vi "Consumer.vi"(8 "error in (no error)":errorcluster, 9 "Data":variant, 10 "Case ID":string, 11 "uService Template in":refnum<class "Common GUI v3.lvclass">) -> (0 "error out":errorcluster, 3 "uService Template out":refnum<class "Common GUI v3.lvclass">)   [LabVIEW 2020, in "TALOS.lvlib" / "Common GUI v3.lvlib" / "Common GUI v3.lvclass"]
uses:
  Common GUI v3.lvclass
  C:/LabVIEW Code/TALOS/talos/Ancestor/Ancestor/Ancestor.lvclass
  Common GUI v3 Consumer Case Selector.ctl
  Classes/Guardian List/Guardian List.lvclass
  Common GUI v3.lvclass/Common GUI v3.ctl
  Ancestor/Ancestor/Ancestor.lvclass/Ancestor.ctl
  Error Listbox Msg.ctl
  Error Listbox Msg Action.ctl
  Error Manager/Error Info.ctl
  Remote uService GUI.ctl
  Classes/uService List/uService List.lvclass/uService List.ctl
  Classes/uService List/Get Remote GUI.vi
  Classes/uService List/Get Remote Window VI Ref.vi
  Classes/uService List/Set Remote Window VI Ref.vi
  Classes/uService List/Get VI Ref.vi
  Support VIs/Generate Error.vi
  FGV/Error Memory/Get Error Description.vi
  Support VIs/Get PC name.vi
  Ancestor/Ancestor/Read ID.vi
  Support VIs/Get Class Name.vi
  <vilib>/Utility/error.llb/Clear Errors.vi
  FGV/Error Memory/Error Memory Core.vi
  <vilib>/AdvancedString/Delimited String to 1D String Array.vi
  Support VIs/Circus Root Path.vi
  FGV/Error Memory/Error Crt Lvl checker.vi
  FGV/Error Memory/Error Memory Core.vi/40c8088d-b597-4017-91af-faa98e00292e.vi
  FGV/Error Memory/Error Memory Core.vi/d4a3ab98-063c-4e44-b43d-fbdcfe6c2be2.vi
  Support VIs/Global Memory.vi
  <vilib>/Utility/LVClass/Get LV Class Name.vi
  Support VIs/Is in Packed Library.vi
  Support VIs/TALOS Root path.vi
  Support VIs/Read CSV worksheet.vi
  Support VIs/Global Constants.vi
  <vilib>/Utility/error.llb/General Error Handler.vi
  Support VIs/Error Log.vi
  Ancestor/Ancestor/Ancestor.lvclass
  <vilib>/Comparison/Equal/Equal Functor/Equal Functor.lvclass
  Classes/uService List/uService List.lvclass
  Father of all uServices/Father of all uServices/Father of all uServices.lvclass
  TALOS.lvlib
  Error Manager/Error Manager.lvclass
  Common GUI v3.lvlib
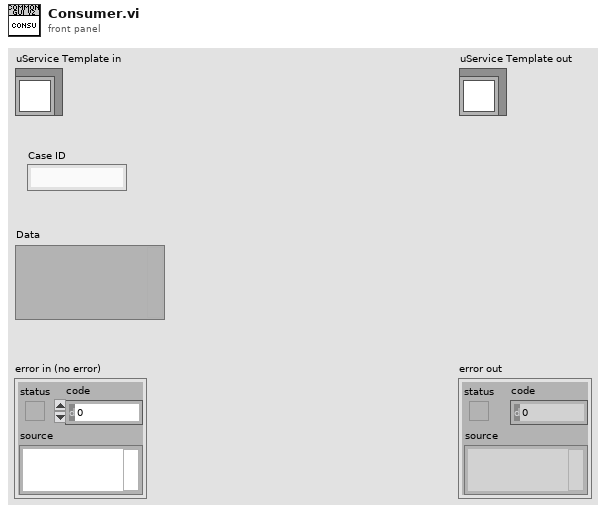
[diagram p1: front panel]
types:
  T1 = typedef "TALOS.lvlib/Common GUI v3.lvlib/Common GUI v3.lvclass/Common GUI v3 Consumer Case Selector.ctl" = enum16{"Update Guardians List", "Update ABORT LED", "Update Guardian ID", "Update Kasli Log", "Update Error Listbox", "Update Run Number", "Change Run LED color", "Update Run Status", "Run Stopped with Errors", "Reset Run LED", "Update Run Config", "Remote GUI"}
  T2 = typedef "TALOS.lvlib/Common GUI v3.lvlib/Common GUI v3.lvclass/Error Listbox Msg.ctl" = cluster{"Action":T3, "Error Info":T4}
  T3 = typedef "TALOS.lvlib/Common GUI v3.lvlib/Common GUI v3.lvclass/Error Listbox Msg Action.ctl" = enum16{"Add", "Remove", "Clear"}
  T4 = typedef "TALOS.lvlib/Error Manager.lvlib/Error Manager.lvclass/Error Info.ctl" = cluster{"error out":errorcluster, "Time Stamp":timestamp, "Machine Name":string, "GUID":string}
  T5 = typedef "TALOS.lvlib/Common GUI v3.lvlib/Remote uService GUI.ctl" = cluster{"Open/Close":bool, "uService ID":string}
  T6 = map{string, cluster{"Online":bool, "Last Poke":timestamp}}
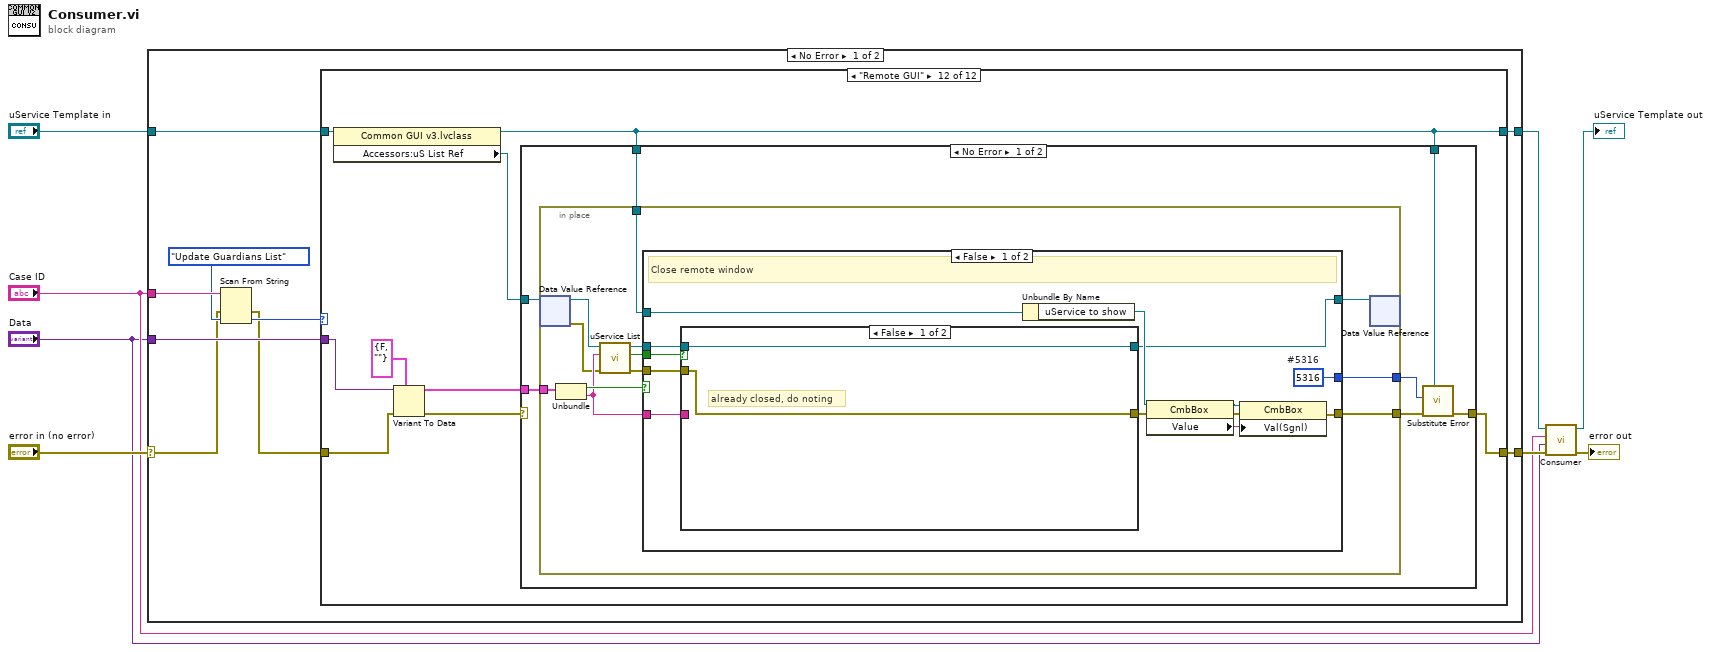
[diagram p0: block diagram]
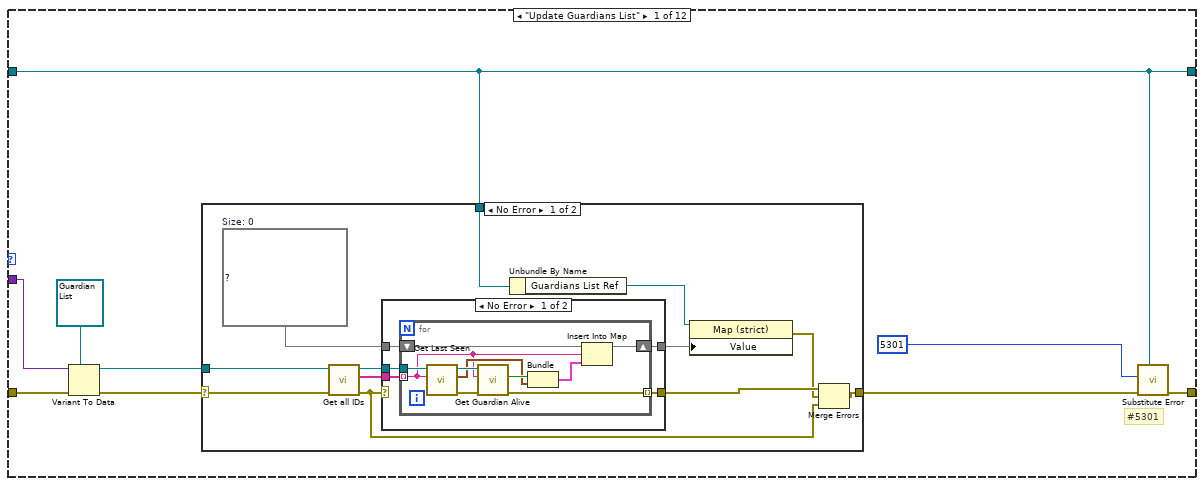
[diagram p2: hidden frame]
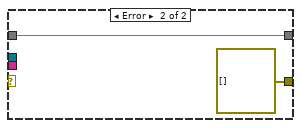
[diagram p3: hidden frame]
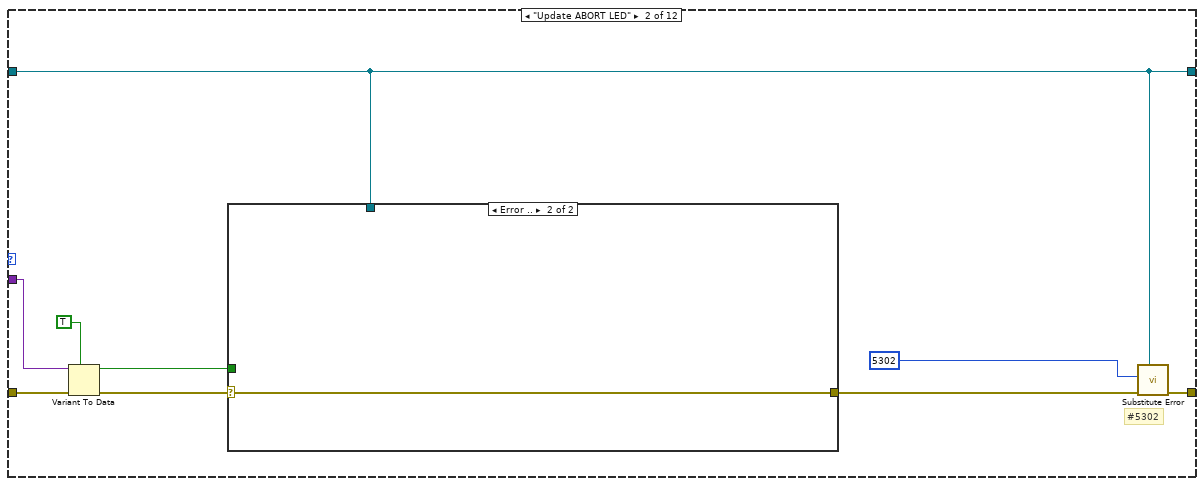
[diagram p5: hidden frame]
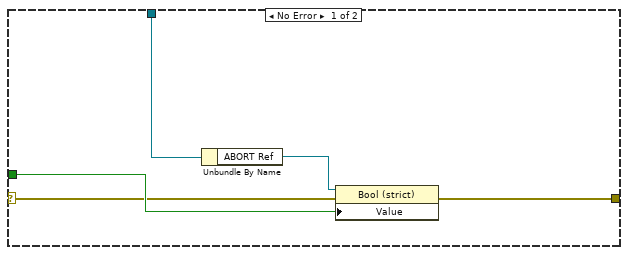
[diagram p6: hidden frame]
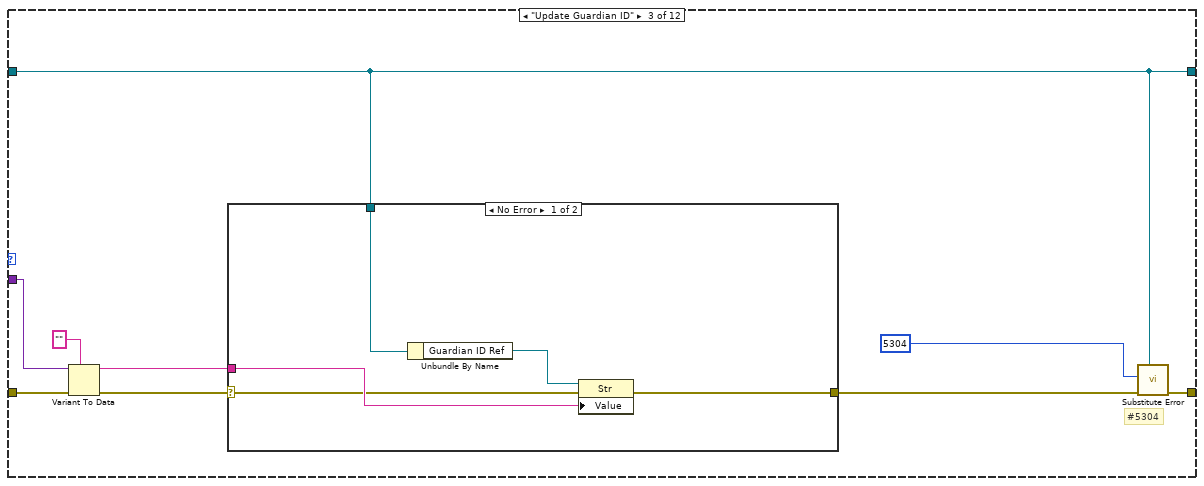
[diagram p7: hidden frame]
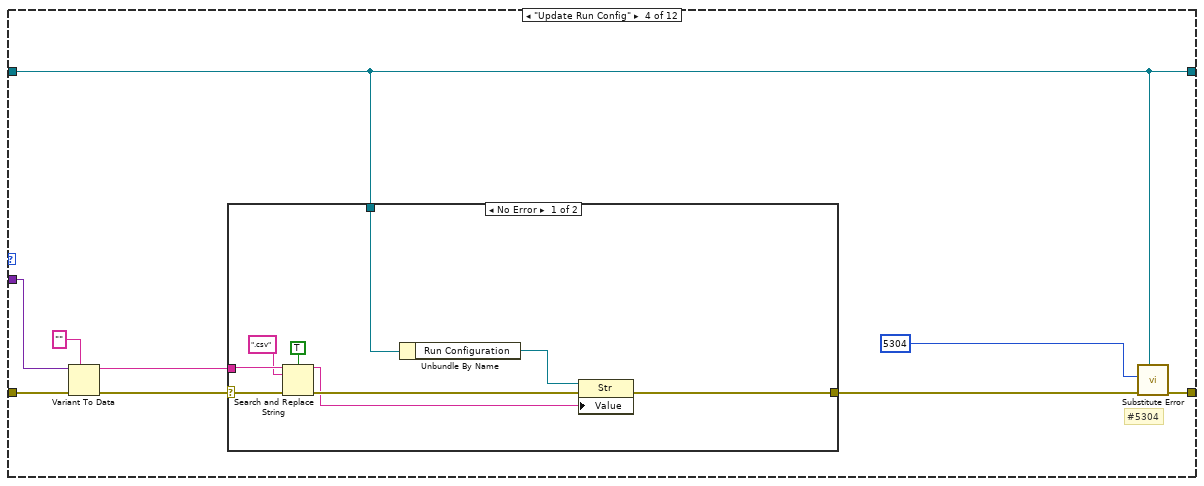
[diagram p9: hidden frame]
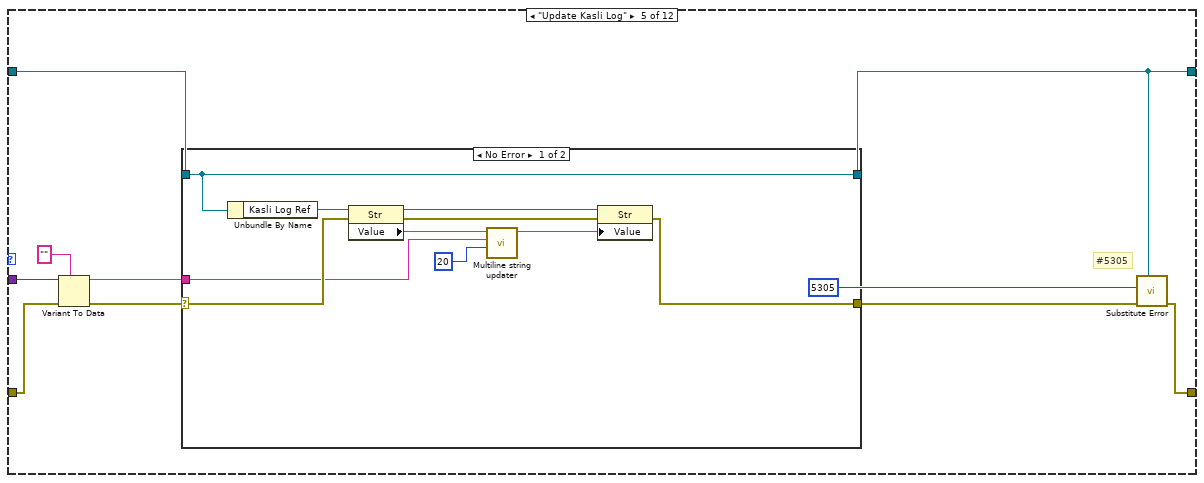
[diagram p11: hidden frame]
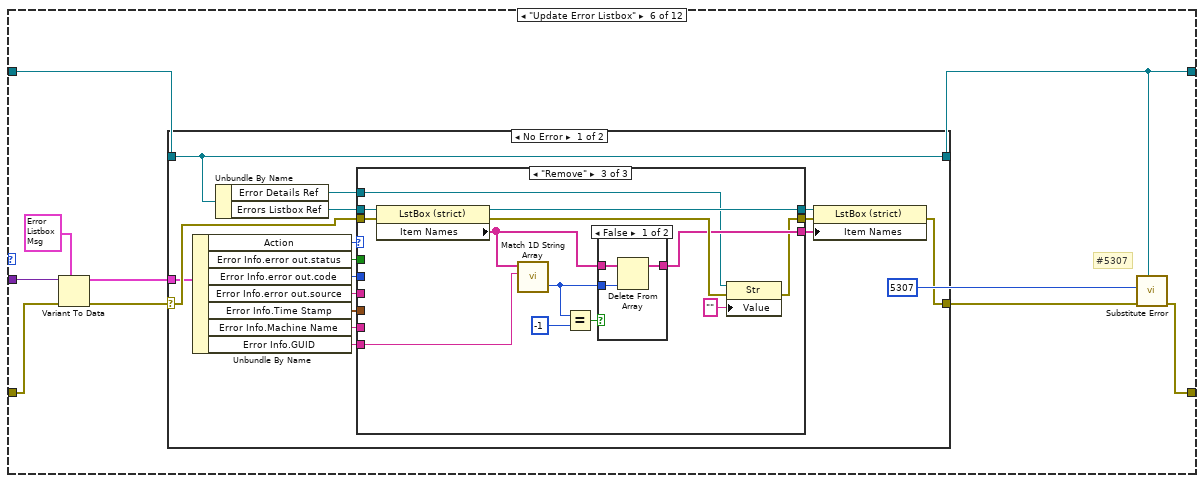
[diagram p13: hidden frame]
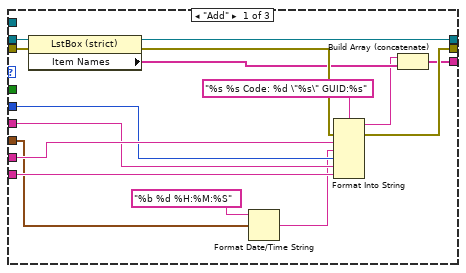
[diagram p14: hidden frame]
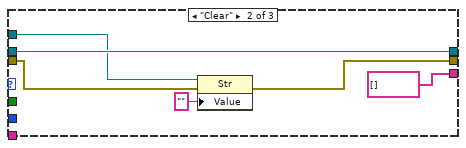
[diagram p15: hidden frame]
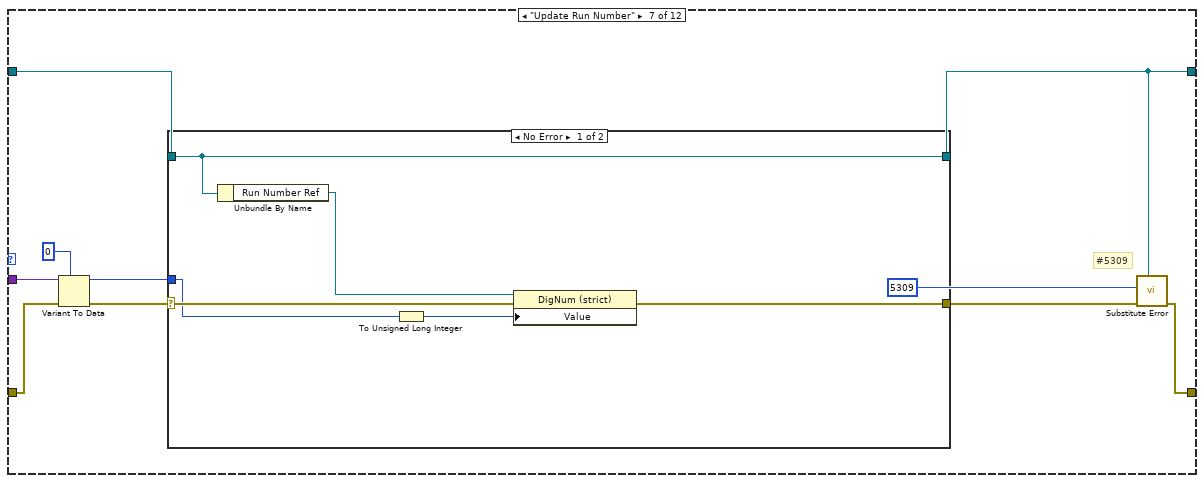
[diagram p18: hidden frame]
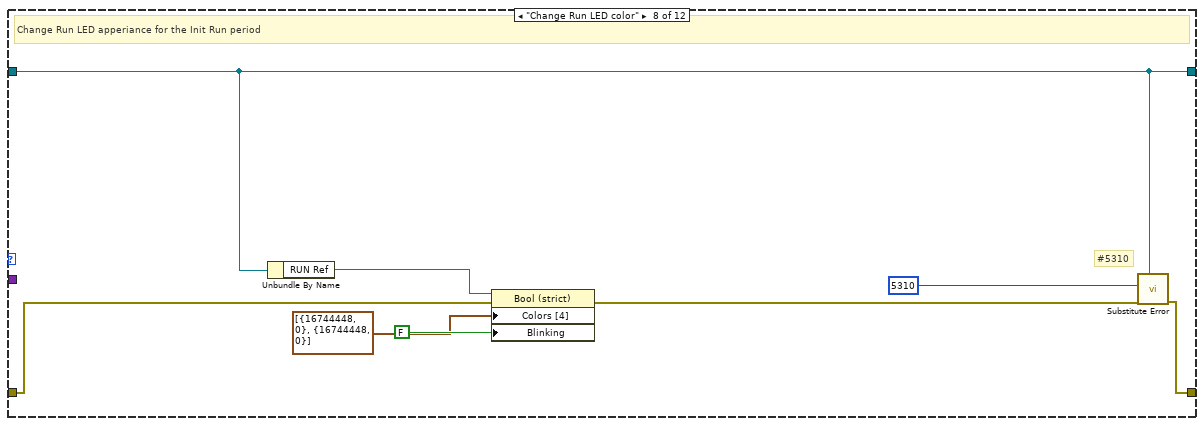
[diagram p20: hidden frame]
diagram:
  n1 = case shown="No Error" "error in (no error)" {
    selector: "error in (no error)" -> [w10 w349]
    tunnel: "uService Template in" -> [w16 w350]
    tunnel: [w14 w350] -> w4
    tunnel: [w15 w349] -> w3
    tunnel: "Case ID" -> [w13 _]
    tunnel: "Data" -> [w17 _]
    frame No Error {
      n2 = Scan From String(input string=w13, error in=w10, default 1=Common_GUI_v3_Consumer_Case_Selector."Update Guardians List") -> (error out=w9:errorcluster, output 1=w11:T1)  [unwired: 2 in, 2 out]
      n3 = case shown="\"Remote GUI\"" w11 {
        tunnel: w17 -> [w23 w63 w78 w93 w114 w136 w203 _ w225 _ _ w257]
        tunnel: w9 -> [w22 w62 w77 w92 w112 w135 w202 w216 w224 _ _ w256]
        tunnel: w16 -> [w19 w59 w74 w89 w115 w137 w204 w217 w226 w240 w246 w254]
        tunnel: [w20 w60 w75 w90 w109 w132 w199 w218 w227 w241 w247 w255] -> w15
        tunnel: [w19 w59 w74 w89 w108 w131 w198 w217 w226 w240 w246 w252] -> w14
        frame "Update Guardians List" {
          # "#5301"
          n4 = Variant To Data(error in=w22, type=refnum<class "Guardian List.lvclass"> refnum ("Guardian List in"), Variant=w23) -> (data=w24:refnum<class "Guardian List.lvclass">, error out=w26:errorcluster)
          n5 = case shown="No Error" w26 {
            selector: w26 -> [w35 w56]
            tunnel: w24 -> [w34 _]
            tunnel: w19 -> [w32 _]
            tunnel: [w29 w56] -> w21
            frame No Error {
              w36 = T6 {}  # Size: 0
              n6 = call-dynamic "Get all IDs.vi"("error in (no error)"=w35, "Guardian List in"=w34) -> ("error out"=w27:errorcluster, "All IDs"=w38:string[], "Guardian List out"=w37:refnum<class "Guardian List.lvclass">)  [unwired: 7 in]
              n7 = case shown="No Error" w27 {
                tunnel: w38 -> [w43 _]
                tunnel: w37 -> [w42 _]
                tunnel: w36 -> [w41 w55]
                tunnel: [w40 errorcluster[] []] -> w33
                tunnel: [w39 w55] -> w30
                frame No Error {
                  n8 = for {
                    tunnel: w43 -> [w47] mode=indexing
                    tunnel: w42 -> [w53]
                    shift-right: [w48] -> w39
                    shift-left: w41 -> [w49]
                    tunnel: [w45] -> w40 mode=indexing
                    n9 = call-dynamic "Get Last Seen.vi"("ID"=w47, "Guardian List in"=w53) -> ("error out"=w44:errorcluster, "Last Poke"=w50:timestamp, "Guardian List out"=w52:refnum<class "Guardian List.lvclass">)  [unwired: 7 in]
                    n10 = call-dynamic "Get Guardian Alive.vi"("error in (no error)"=w44, "ID"=w47, "Guardian List in"=w52) -> ("error out"=w45:errorcluster, "Alive"=w51:bool)  [unwired: 6 in, 1 out]
                    n11 = Bundle("Alive"=w51, "Last Poke"=w50) -> (w46:cluster{"Alive":bool, "Last Poke":timestamp})  [unwired: 1 in]
                    n12 = Insert Into Map(map in=w49, key=w47, value=w46) -> (map out=w48:T6)  [unwired: 2 out]
                  }
                }
                frame Error {
                }
              }
              n13 = Unbundle By Name(w32) -> ("Guardians List Ref"=w31:refnum<vi>)
              n14 = property class="Map (strict)"(reference=w31, "Value"=w30) -> (error out=w28:errorcluster)  [unwired: 1 in, 1 out]
              n15 = Merge Errors(w33, w28, w27) -> (w29:errorcluster)
            }
            frame Error {
            }
          }
          n16 = call "Substitute Error.vi"("LabVIEW Object"=w19, "error in (no error)"=w21, "Error Code"=5301) -> ("error out"=w20:errorcluster)  [unwired: 8 in]
        }
        frame "Update ABORT LED" {
          # "#5302"
          n17 = Variant To Data(error in=w62, type=TRUE, Variant=w63) -> (data=w64:bool, error out=w65:errorcluster)
          n18 = case shown="Error .." w65 {
            selector: w65 -> [w67 w71]
            tunnel: w64 -> [w68 _]
            tunnel: w59 -> [w70 _]
            tunnel: [w69 w71] -> w61
            frame No Error {
              n19 = Unbundle By Name(w70) -> ("ABORT Ref"=w66:refnum<vi>)
              n20 = property class="Bool (strict)"(reference=w66, error in=w67, "Value"=w68) -> (error out=w69:errorcluster)  [unwired: 1 out]
            }
            frame Error {
            }
          }
          n21 = call "Substitute Error.vi"("LabVIEW Object"=w59, "error in (no error)"=w61, "Error Code"=5302) -> ("error out"=w60:errorcluster)  [unwired: 8 in]
        }
        frame "Update Guardian ID" {
          # "#5304"
          n22 = Variant To Data(error in=w77, type="", Variant=w78) -> (data=w79:string, error out=w80:errorcluster)
          n23 = case shown="No Error" w80 {
            selector: w80 -> [w82 w86]
            tunnel: w79 -> [w83 _]
            tunnel: w74 -> [w85 _]
            tunnel: [w84 w86] -> w76
            frame No Error {
              n24 = Unbundle By Name(w85) -> ("Guardian ID Ref"=w81:refnum<vi>)
              n25 = property class="Str"(reference=w81, error in=w82, "Value"=w83) -> (error out=w84:errorcluster)  [unwired: 1 out]
            }
            frame Error {
            }
          }
          n26 = call "Substitute Error.vi"("LabVIEW Object"=w74, "error in (no error)"=w76, "Error Code"=5304) -> ("error out"=w75:errorcluster)  [unwired: 8 in]
        }
        frame "Update Run Config" {
          # "#5304"
          n27 = Variant To Data(error in=w92, type="", Variant=w93) -> (data=w94:string, error out=w95:errorcluster)
          n28 = case shown="No Error" w95 {
            selector: w95 -> [w101 w105]
            tunnel: w94 -> [w99 _]
            tunnel: w89 -> [w104 _]
            tunnel: [w103 w105] -> w91
            frame No Error {
              n29 = Search and Replace String(case sensitive?=TRUE ("ignore case? (F)"), input string=w99, search string=".csv", error in=w101) -> (result string=w96:string, error out=w100:errorcluster)  [unwired: 4 in, 2 out]
              n30 = Unbundle By Name(w104) -> ("Run Configuration"=w102:refnum<vi>)
              n31 = property class="Str"(reference=w102, error in=w100, "Value"=w96) -> (error out=w103:errorcluster)  [unwired: 1 out]
            }
            frame Error {
            }
          }
          n32 = call "Substitute Error.vi"("LabVIEW Object"=w89, "error in (no error)"=w91, "Error Code"=5304) -> ("error out"=w90:errorcluster)  [unwired: 8 in]
        }
        frame "Update Kasli Log" {
          # "#5305"
          n33 = Variant To Data(error in=w112, type="", Variant=w114) -> (data=w106:string, error out=w111:errorcluster)
          n34 = case shown="No Error" w111 {
            selector: w111 -> [w124 w126]
            tunnel: w115 -> [w116 w127]
            tunnel: [w116 w127] -> w108
            tunnel: [w117 w126] -> w110
            tunnel: w106 -> [w119 _]
            frame No Error {
              n35 = Unbundle By Name(w116) -> ("Kasli Log Ref"=w125:refnum<vi>)
              n36 = property class="Str"(reference=w125, error in=w124) -> (reference out=w123:refnum<vi>, error out=w122:errorcluster, "Value"=w121:string)
              n37 = call "Multiline string updater.vi"("Lines to keep"=u8 20, "String to add"=w119, "Multiline string in"=w121) -> ("Multiline string out"=w120:string)  [unwired: 8 in]
              n38 = property class="Str"(reference=w123, error in=w122, "Value"=w120) -> (error out=w117:errorcluster)  [unwired: 1 out]
            }
            frame Error {
            }
          }
          n39 = call "Substitute Error.vi"("LabVIEW Object"=w108, "error in (no error)"=w110, "Error Code"=5305) -> ("error out"=w109:errorcluster)  [unwired: 8 in]
        }
        frame "Update Error Listbox" {
          # "#5307"
          n40 = Variant To Data(error in=w135, type=T2 {"Action"=enum."Add", "Error Info"={"error out"={"status"=FALSE, "code"=0, "source"=""}, "Time Stamp"=timestamp(0 s since 1904-01-01), "Machine Name"="", "GUID"=""}} ("Error Listbox Msg"), Variant=w136) -> (data=w129:T2, error out=w134:errorcluster)
          n41 = case shown="No Error" w134 {
            selector: w134 -> [w152 w193]
            tunnel: w137 -> [w151 w194]
            tunnel: [w151 w194] -> w131
            tunnel: [w139 w193] -> w133
            tunnel: w129 -> [w150 _]
            frame No Error {
              n42 = Unbundle By Name(w150) -> ("Action"=w149:T3, "Error Info.error out.status"=w148:bool, "Error Info.error out.code"=w147:i32, "Error Info.error out.source"=w146:string, "Error Info.Time Stamp"=w145:timestamp, "Error Info.Machine Name"=w144:string, "Error Info.GUID"=w143:string)
              n43 = Unbundle By Name(w151) -> ("Error Details Ref"=w138:refnum<vi>, "Errors Listbox Ref"=w153:refnum<vi>)
              n44 = case shown="\"Remove\"" w149 {
                tunnel: w153 -> [w169 w175 w187]
                tunnel: w152 -> [w168 w172 w186]
                tunnel: w148 -> [_ _ _]
                tunnel: w147 -> [w162 _ _]
                tunnel: w146 -> [w161 _ _]
                tunnel: w145 -> [w155 _ _]
                tunnel: w144 -> [w164 _ _]
                tunnel: w143 -> [w160 _ w182]
                tunnel: [w159 w175 w185] -> w142
                tunnel: [w158 w171 w176] -> w141
                tunnel: [w157 string[] [] ("Item Names") w184] -> w140
                tunnel: w138 -> [_ w173 w177]
                frame "Add" {
                  n45 = property class="LstBox (strict)"(reference=w169, error in=w168) -> (reference out=w159:refnum<vi>, error out=w167:errorcluster, "Item Names"=w166:string[])
                  n46 = Format Date/Time String(time format string (%c)="%b %d %H:%M:%S", seconds (now)=w155) -> (date/time string=w154:string)  [unwired: 1 in]
                  n47 = Format Into String(format string="%s %s Code: %d \"%s\" GUID:%s", error in=w167, w164, w154, w162, w161, w160) -> (resulting string=w165:string, error out=w158:errorcluster)  [unwired: 1 in]
                  n48 = Build Array (concatenate)(w165, w166) -> (w157:string[])
                }
                frame "Clear" {
                  n49 = property class="Str"(reference=w173, error in=w172, "Value"="") -> (error out=w171:errorcluster)  [unwired: 1 out]
                }
                frame "Remove" {
                  n50 = property class="LstBox (strict)"(reference=w187, error in=w186) -> (reference out=w185:refnum<vi>, error out=w188:errorcluster, "Item Names"=w183:string[])
                  n51 = call <vilib>:"Match 1D String Array.vi"("Pattern"=w182, "Strings"=w183) -> ("index of element"=w180:i32)  [unwired: 2 in, 1 out]
                  n52 = Equal?(x=w180, y=-1) -> (x = y?=w179:bool)
                  n53 = case shown="False" w179 {
                    tunnel: [w191 w192] -> w184
                    tunnel: w183 -> [w190 w192]
                    tunnel: w180 -> [w189 _]
                    frame False {
                      n54 = Delete From Array(array=w190, index=w189) -> (array with subset deleted=w191:string[])  [unwired: 1 in, 1 out]
                    }
                    frame True {
                      # "Not found!"
                    }
                  }
                  n55 = property class="Str"(reference=w177, error in=w188, "Value"="") -> (error out=w176:errorcluster)  [unwired: 1 out]
                }
              }
              n56 = property class="LstBox (strict)"(reference=w142, error in=w141, "Item Names"=w140) -> (error out=w139:errorcluster)  [unwired: 1 out]
            }
            frame Error {
            }
          }
          n57 = call "Substitute Error.vi"("LabVIEW Object"=w131, "error in (no error)"=w133, "Error Code"=5307) -> ("error out"=w132:errorcluster)  [unwired: 8 in]
        }
        frame "Update Run Number" {
          # "#5309"
          n58 = Variant To Data(error in=w202, type=0, Variant=w203) -> (data=w196:i32, error out=w201:errorcluster)
          n59 = case shown="No Error" w201 {
            selector: w201 -> [w207 w211]
            tunnel: w204 -> [w210 w212]
            tunnel: [w210 w212] -> w198
            tunnel: [w209 w211] -> w200
            tunnel: w196 -> [w205 _]
            frame No Error {
              n60 = Unbundle By Name(w210) -> ("Run Number Ref"=w208:refnum<vi>)
              n61 = To Unsigned Long Integer(number=w205) -> (unsigned 32bit integer=w206:u32)
              n62 = property class="DigNum (strict)"(reference=w208, error in=w207, "Value"=w206) -> (error out=w209:errorcluster)  [unwired: 1 out]
            }
            frame Error {
            }
          }
          n63 = call "Substitute Error.vi"("LabVIEW Object"=w198, "error in (no error)"=w200, "Error Code"=5309) -> ("error out"=w199:errorcluster)  [unwired: 8 in]
        }
        frame "Change Run LED color" {
          # "#5310"
          # "Change Run LED apperiance for the Init Run period"
          n64 = Unbundle By Name(w217) -> ("RUN Ref"=w214:refnum<vi>)
          n65 = property class="Bool (strict)"(reference=w214, error in=w216, "Colors [4]"=cluster{u32, u32}[] [{16744448, 0}, {16744448, 0}], "Blinking"=FALSE) -> (error out=w219:errorcluster)  [unwired: 1 out]
          n66 = call "Substitute Error.vi"("LabVIEW Object"=w217, "error in (no error)"=w219, "Error Code"=5310) -> ("error out"=w218:errorcluster)  [unwired: 8 in]
        }
        frame "Update Run Status" {
          # "#5310"
          n67 = Variant To Data(error in=w224, type=TRUE, Variant=w225) -> (data=w221:bool, error out=w223:errorcluster)
          n68 = case shown="No Error" w223 {
            selector: w223 -> [w232 w236]
            tunnel: [w235 w236] -> w229
            tunnel: w226 -> [w233 _]
            tunnel: w221 -> [w231 _]
            frame No Error {
              n69 = Unbundle By Name(w233) -> ("RUN Ref"=w234:refnum<vi>)
              n70 = property class="Bool (strict)"(reference=w234, error in=w232, "Value"=w231, "Colors [4]"=cluster{u32, u32}[] [{160, 0}, {6618880, 0}]) -> (error out=w235:errorcluster)  [unwired: 1 out]
            }
            frame Error {
            }
          }
          n71 = call "Substitute Error.vi"("LabVIEW Object"=w226, "error in (no error)"=w229, "Error Code"=5310) -> ("error out"=w227:errorcluster)  [unwired: 8 in]
        }
        frame "Run Stopped with Errors" {
          # "#5310"
          n72 = Unbundle By Name(w240) -> ("RUN Ref"=w244:refnum<vi>)
          n73 = property class="Bool (strict)"(reference=w244, "Blinking"=TRUE, "Value"=FALSE, "Colors [4]"=cluster{u32, u32}[] [{160, 0}, {6618880, 0}] ("Colors")) -> (error out=w242:errorcluster)  [unwired: 1 in, 1 out]
          n74 = call "Substitute Error.vi"("LabVIEW Object"=w240, "error in (no error)"=w242, "Error Code"=5310) -> ("error out"=w241:errorcluster)  [unwired: 8 in]
        }
        frame "Reset Run LED" {
          # "#5310"
          n75 = Unbundle By Name(w246) -> ("RUN Ref"=w251:refnum<vi>)
          n76 = property class="Bool (strict)"(reference=w251, "Blinking"=FALSE, "Colors [4]"=cluster{u32, u32}[] [{160, 0}, {6618880, 0}] ("Colors")) -> (error out=w248:errorcluster)  [unwired: 1 in, 1 out]
          n77 = call "Substitute Error.vi"("LabVIEW Object"=w246, "error in (no error)"=w248, "Error Code"=5310) -> ("error out"=w247:errorcluster)  [unwired: 8 in]
        }
        frame "Remote GUI" {
          n78 = property class="Common GUI v3.lvclass"(reference=w254) -> (reference out=w252:refnum<class "Common GUI v3.lvclass">, "Accessors:uS List Ref"=w253:refnum<data-value>)  [unwired: 1 in, 1 out]
          n79 = Variant To Data(error in=w256, type=T5 {"Open/Close"=FALSE, "uService ID"=""} ("Remote GUI"), Variant=w257) -> (data=w258:T5, error out=w259:errorcluster)
          n80 = case shown="No Error" w259 {
            selector: w259 -> [_ w348]
            tunnel: w258 -> [w267 _]
            tunnel: [w266 w347] -> w255
            tunnel: w252 -> [w263 w345]
            tunnel: w253 -> [w262 _]
            tunnel: w252 -> [w261 _]
            frame No Error {
              n81 = in-place {
                in-place-border: w267 -> [w279]
                in-place-border: [w273] -> w265
                in-place-border: [w272] -> w264
                in-place-border: w261 -> [w269]
                n82 = in-place-dvr #1(w262) -> (w271:refnum<class "uService List.lvclass">, w270:errorcluster)
                n83 = Unbundle(w279) -> ("Open/Close"=w278:bool, "uService ID"=w275:string)
                n84 = call-poly "uService List.vi"("error in (no error)"=w270, "ID"=w275, "uService List in"=w271) -> ("error out"=w274:errorcluster, "Remote GUI"=w276:bool, "uService List out"=w277:refnum<class "uService List.lvclass">)  [unwired: 6 in]
                n85 = case shown="False" w278 {
                  tunnel: w277 -> [w291 w320]
                  tunnel: w276 -> [w292 w321]
                  tunnel: w275 -> [w289 w319]
                  tunnel: w274 -> [w290 w318]
                  tunnel: [w287 w317] -> w273
                  tunnel: w269 -> [w281 w316]
                  tunnel: [w288 w315] -> w272
                  tunnel: [w280 w314] -> w268
                  frame False {
                    w288 = 5316  # #5316
                    # "Close remote window"
                    n86 = case shown="False" w292 {
                      tunnel: w291 -> [w293 w307]
                      tunnel: w290 -> [w294 w306]
                      tunnel: w289 -> [_ w303]
                      tunnel: [w294 w296] -> w286
                      tunnel: [w293 w295] -> w280
                      frame False {
                        # "already closed, do noting"
                      }
                      frame True {
                        n87 = call-poly "uService List.vi"("error in (no error)"=w306, "ID"=w303, "uService List in"=w307) -> ("error out"=w302:errorcluster, "Vi Ref"=w304:refnum<vi>, "uService List out"=w305:refnum<class "uService List.lvclass">)  [unwired: 6 in]
                        n88 = call "Close Remote uService GUI.vi"("error in (no error)"=w302, "Remote GUI"=w304) -> ("error out"=w301:errorcluster, "reference out"=w300:refnum<vi>)  [unwired: 8 in]
                        n89 = case shown="No Error" w301 {
                          selector: w301 -> [w308 w310]
                          tunnel: w300 -> [_ w313]
                          tunnel: [w308 w309] -> w297
                          frame No Error {
                          }
                          frame Error {
                            n90 = invoke class="VI" method="Abort VI"(reference=w313, error in=w310) -> (reference out=w312:refnum<vi>, error out=w311:errorcluster)  [unwired: 1 in, 1 out]
                            n91 = invoke class="VI" method="FP.Close"(reference=w312, error in=w311) -> (error out=w309:errorcluster)  [unwired: 1 in, 2 out]
                          }
                        }
                        n92 = call-poly "uService List.vi"("Vi Ref"=refnum<vi> refnum, "ID"=w303, "uService List in"=w305) -> ("error out"=w298:errorcluster, "uService List out"=w295:refnum<class "uService List.lvclass">)  [unwired: 7 in]
                        n93 = Merge Errors(w298, w297) -> (w296:errorcluster)
                      }
                    }
                    n94 = Unbundle By Name(w281) -> ("uService to show"=w283:refnum<vi>)
                    n95 = property class="CmbBox"(reference=w283, error in=w286) -> (reference out=w282:refnum<vi>, error out=w284:errorcluster, "Value"=w285:string)
                    n96 = property class="CmbBox"(reference=w282, error in=w284, "Val(Sgnl)"=w285) -> (error out=w287:errorcluster)  [unwired: 1 out]
                  }
                  frame True {
                    w315 = 5315  # #5315
                    # "Open remote window"
                    n97 = case shown="False" w321 {
                      tunnel: w320 -> [w327 w343]
                      tunnel: w319 -> [w325 w339]
                      tunnel: w318 -> [w326 w344]
                      tunnel: [w331 w338] -> w317
                      tunnel: w316 -> [w330 _]
                      tunnel: [w322 w337] -> w314
                      frame False {
                        n98 = Unbundle By Name(w330) -> ("Sub Panel Reference"=w329:refnum<vi>)
                        n99 = call-poly "uService List.vi"("error in (no error)"=w326, "ID"=w325, "uService List in"=w327) -> ("error out"=w336:errorcluster, "Vi Ref"=w324:refnum<vi>, "uService List out"=w323:refnum<class "uService List.lvclass">)  [unwired: 6 in]
                        n100 = invoke class="SubPnl" method="Remove VI"(reference=w329, error in=w336) -> (error out=w328:errorcluster)  [unwired: 1 in, 2 out]
                        n101 = call "Open Remote uService GUI.vi"("error in (no error)"=w328, "GUI VI"=w324, "uService ID"=w325, "Message Enqueuer"=w330) -> ("error out"=w333:errorcluster, "Remote GUI ref"=w335:refnum<vi>, "uService ID dup"=w332:string)  [unwired: 5 in]
                        n102 = call-poly "uService List.vi"("Vi Ref"=w335, "ID"=w332, "uService List in"=w323) -> ("error out"=w334:errorcluster, "uService List out"=w322:refnum<class "uService List.lvclass">)  [unwired: 7 in]
                        n103 = Merge Errors(w334, w333) -> (w331:errorcluster)
                      }
                      frame True {
                        n104 = call-poly "uService List.vi"("error in (no error)"=w344, "ID"=w339, "uService List in"=w343) -> ("error out"=w341:errorcluster, "Vi Ref"=w342:refnum<vi>, "uService List out"=w337:refnum<class "uService List.lvclass">)  [unwired: 6 in]
                        n105 = property class="VI"(reference=w342, error in=w341, "Front Panel.IsFrontmost"=TRUE ("Front Panel Window:Is Frontmost")) -> (error out=w338:errorcluster)  [unwired: 1 out]
                      }
                    }
                  }
                }
                n106 = in-place-dvr #1(w268) -> ()  [unwired: 2 out]
              }
              n107 = call "Substitute Error.vi"("LabVIEW Object"=w263, "error in (no error)"=w265, "Error Code"=w264) -> ("error out"=w266:errorcluster)  [unwired: 8 in]
            }
            frame Error {
              w346 = 5317  # #5317
              n108 = call "Substitute Error.vi"("LabVIEW Object"=w345, "error in (no error)"=w348, "Error Code"=w346) -> ("error out"=w347:errorcluster)  [unwired: 8 in]
            }
          }
        }
      }
    }
    frame Error {
    }
  }
  n109 = call-parent "Consumer.vi"("error in (no error)"=w3, "Data"="Data", "Case ID"="Case ID", "uService Template in"=w4) -> ("error out"=→"error out":errorcluster, "uService Template out"=→"uService Template out":refnum<class "Common GUI v3.lvclass">)  [unwired: 6 in]
